vi "start Julia ZMQ server.vi"(8 "error in (no error)":errorcluster, 11 "Julia user functions script":path=path "C:/_LabView_projects/ZMQ/LV_ZMQ_Jl.jl/src/Julia/dummy.jl") -> (0 "error out":errorcluster, 1 "tmp file out":path, 2 "jl-script file out":path, 3 "return code":i32)   [LabVIEW 2018, in "LV2Julia_core.lvlib"]
uses:
  LV2Julia_core.lvlib
  jl-scripts path.vi
  <vilib>/ErrorRing/Error Ring.xnode
  <vilib>/Utility/error.llb/Error Cluster From Error Code.vi
panel:
  out "Julia script":string
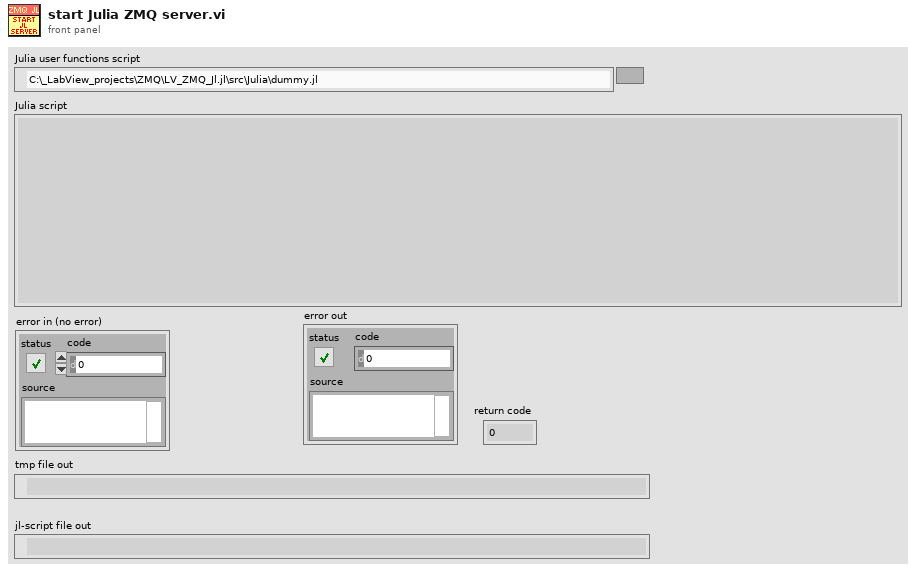
[diagram p1: front panel]
types:
  T1 = enum16{"open", "replace", "create", "open or create", "replace or create", "replace or create with confirmation"}
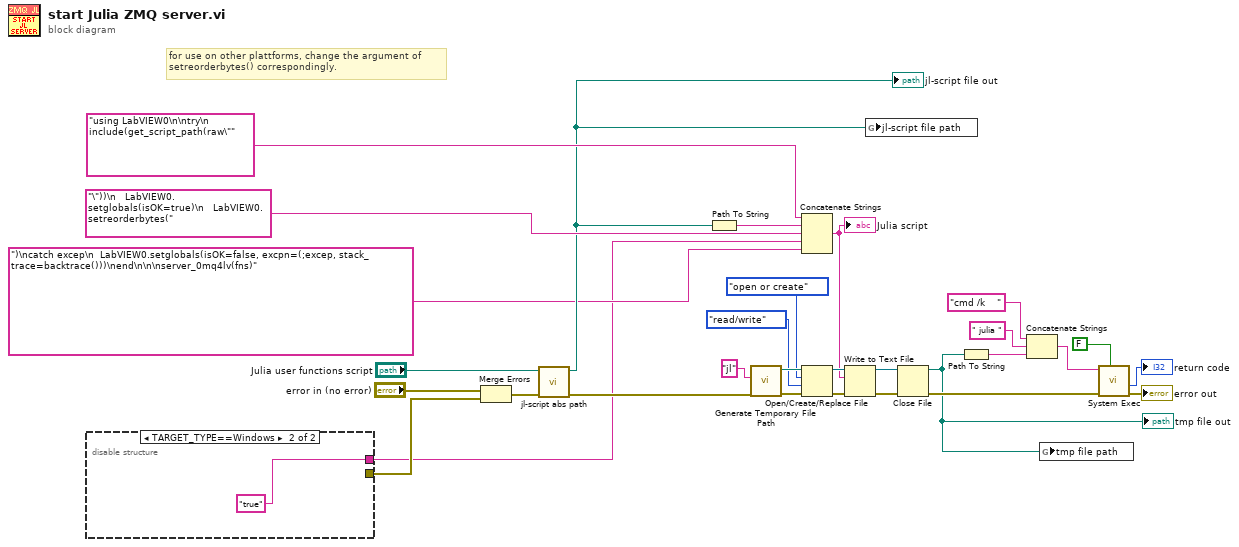
[diagram p0: block diagram]
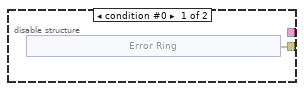
[diagram p2: hidden frame]
diagram:
  # "for use on other plattforms, change the argument of\nsetreorderbytes() correspondingly."
  n1 = disable-structure shown="TARGET_TYPE==Windows" {
    disable-tunnel: [_ "true"] -> w1
    disable-tunnel: [w31 _] -> w2
    frame condition #0 {
      n2 = xnode "Error Ring"() -> ("error out"=w31:errorcluster)
    }
    frame condition #1 (active) {
    }
  }
  n3 = Merge Errors("error in (no error)", w2) -> (w3:errorcluster)
  n4 = call "jl-script abs path.vi"("error in (no error)"=w3, "Julia user functions script"="Julia user functions script") -> ("error out"=w9:errorcluster, "script abs path"=w6:path)  [unwired: 8 in]
  "jl-script file out" <- w6
  n5 = Path To String(path=w6) -> (string=w5:string)
  n6 = call <vilib>:"Generate Temporary File Path.vi"("error in (no error)"=w9, "Temporary File Extension (tmp)"="jl") -> ("error out"=w26:errorcluster, "Unique Temporary File Path"=w27:path)  [unwired: 8 in]
  n7 = Concatenate Strings("using LabVIEW0\n\ntry\n   include(get_script_path(raw\"", w5, "\"))\n   LabVIEW0.setglobals(isOK=true)\n   LabVIEW0.setreorderbytes(", w1, ")\ncatch excep\n  LabVIEW0.setglobals(isOK=false, excpn=(;excep, stack_trace=backtrace()))\nend\n\n\nserver_0mq4lv(fns)") -> (w21:string)
  "Julia script" <- w21
  n8 = Open/Create/Replace File(file path (use dialog)=w27, error in=w26, operation (0:open)=T1."open or create", access (0:read/write)=enum16{"read/write", "read-only", "write-only"}."read/write") -> (refnum out=w22:refnum<file>, error out=w23:errorcluster)  [unwired: 2 in, 1 out]
  n9 = Write to Text File(file (use dialog)=w22, text=w21, error in=w23) -> (refnum out=w20:refnum<file>, error out=w19:errorcluster)  [unwired: 1 in, 1 out]
  n10 = global write "jl-scripts path.vi" "jl-script file path"(w6) -> ()
  n11 = Close File(refnum=w20, error in=w19) -> (path=w8:path, error out=w11:errorcluster)
  "tmp file out" <- w8
  n12 = Path To String(path=w8) -> (string=w15:string)
  n13 = Concatenate Strings("cmd /k    ", " julia ", w15) -> (w14:string)
  n14 = global write "jl-scripts path.vi" "tmp file path"(w8) -> ()
  n15 = call <vilib>:"System Exec.vi"("wait until completion? (T)"=FALSE, "error in (no error)"=w11, "command line"=w14) -> ("error out"=→"error out":errorcluster, "return code"=→"return code":i32)  [unwired: 5 in, 2 out]
